vi "Get Tree Items.vi"(8 "Control.Label":string, 9 "VIs.Ctrls":T4[](array[typedef]), 10 "FP.Tr":map{string, T1}(c390), 11 "Data":T6) -> (0 "Used CTRL":bool, 1 "Caption.Visible":bool, 2 "Selected CTRLs":T4[](array[typedef]), 3 "Use in VIs":string[](array[string]), 4 "Tree Items":T7(array[cluster]), 5 "Class Name":T5, 7 "Comment":string)   [LabVIEW 2019, in "Language Editor.lvlib"]
doc: "- - -\nCopyright (c) 2026, Merecs Engineering GmbH"
uses:
  Language Editor.lvlib
  Language Selection/community/Cluster Settings Data.ctl
  type defs/Cluster VI controls.ctl
  type defs/Enum Class Name.ctl
  type defs/Cluster Translations.ctl
  Language Selection/TypeDefs/Cluster PropertyTranslation.ctl
  Language Selection/TypeDefs/Enum Property Type.ctl
  Language Selection/Language Selection.lvlib
panel:
  # "Connector Pane"
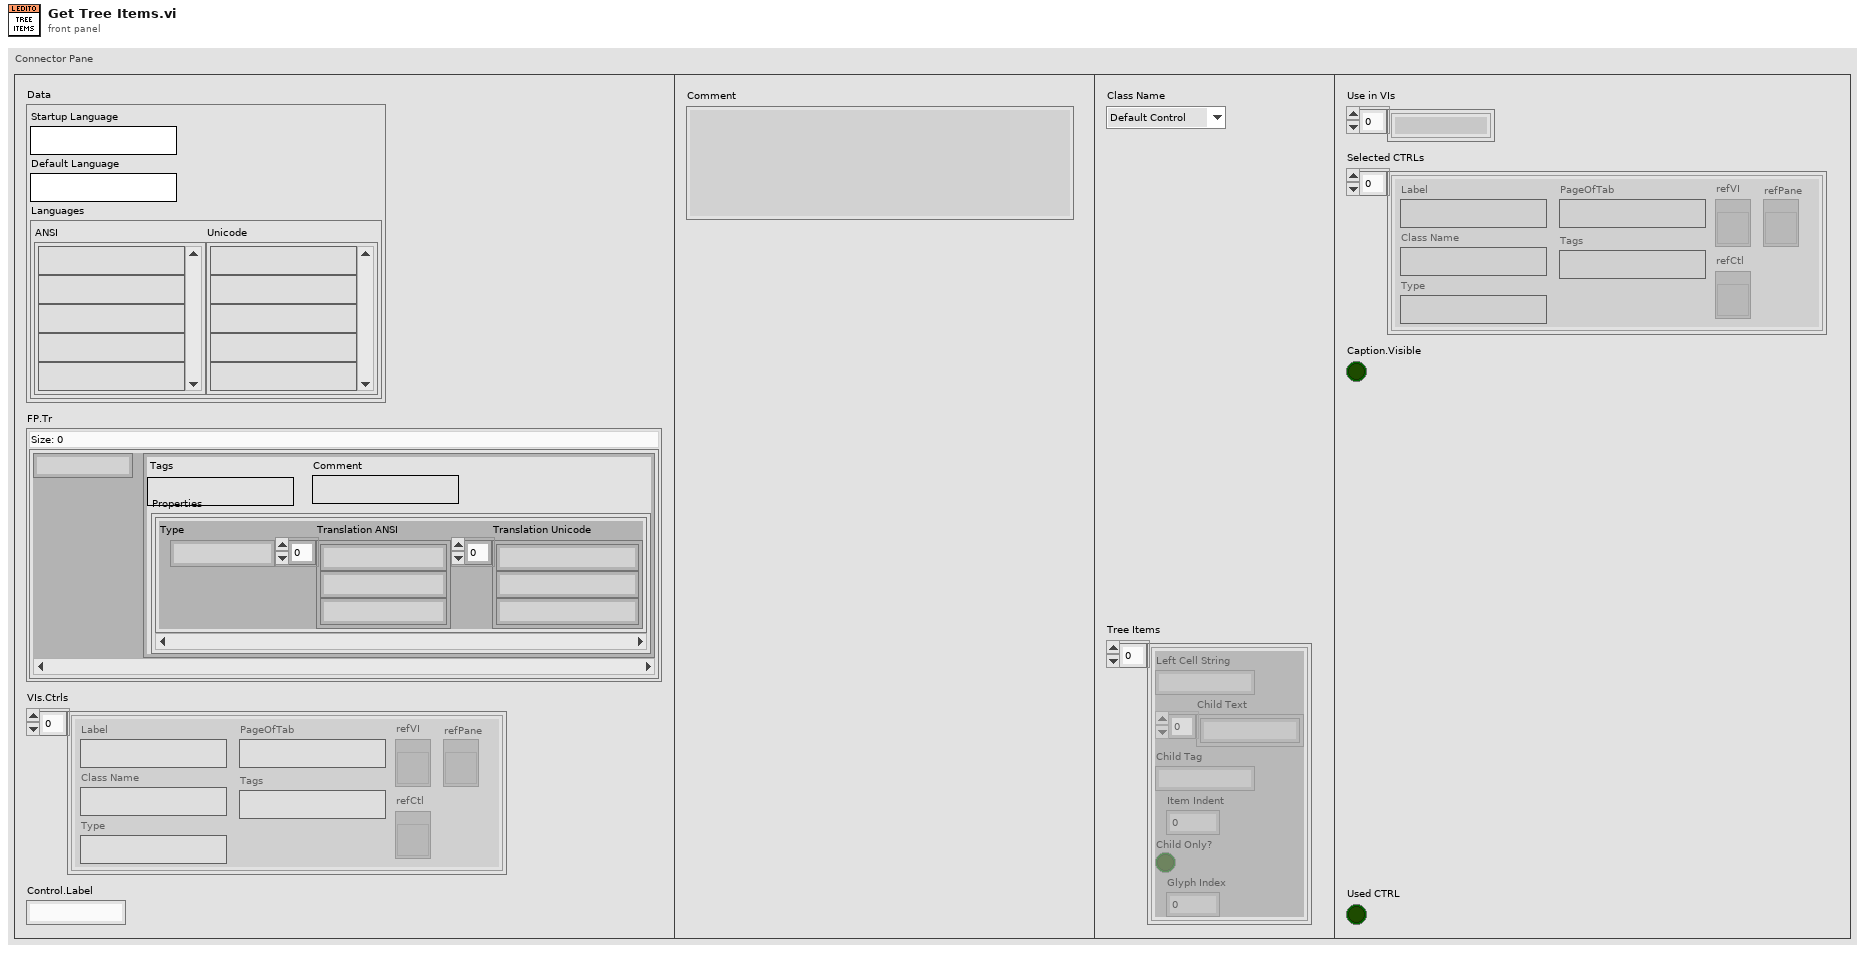
[diagram p1: front panel]
types:
  T1 = typedef "Language Editor.lvlib/Cluster Translations.ctl" = cluster{"Tags":string, "Comment":string, "Properties":T2[]}
  T2 = typedef "Language Selection.lvlib/Cluster PropertyTranslation.ctl" = cluster{"Type":T3, "Translation ANSI":string[], "Translation Unicode":string[]}
  T3 = typedef "Language Selection.lvlib/Enum Property Type.ctl" = enum16{"NA", "Caption", "String Value", "Boolean Text", "Ring Strings", "1D Array Elements", "2D Array Elements", "(MC)Listbox Header", "(MC)Listbox Items", "Tab Pages Names", "X & Y GraphChart", "Plot Names", "Table Headers", "Table Items", "TipStrip", "Combobox Strings", "Cursor Name", "Tree Col Headers"}
  T4 = typedef "Language Editor.lvlib/Cluster VI controls.ctl" = cluster{"Label":string, "Class Name":string, "Type":string, "Tags":string, "refVI":refnum<vi>, "refCtl":refnum<vi>, "PageOfTab":string, "refPane":refnum<vi>}
  T5 = typedef "Language Editor.lvlib/Enum Class Name.ctl" = enum16{"Default Control", "Boolean", "ListBox", "Table", "Graph", "Array", "Ring", "String", "TabControl", "ComboBox", "TreeControl"}
  T6 = typedef "Language Selection.lvlib/Cluster Settings Data.ctl" = cluster{"Startup Language":string, "Default Language":string, "Languages":cluster{"ANSI":string[], "Unicode":string[]}}
  T7 = cluster{"Left Cell String":string, "Child Text":string[], "Child Tag":string, "Item Indent":i32, "Child Only?":bool, "Glyph Index":i32}[]
  T8 = cluster{"Left Cell String":string, "Child Text":string[], "Child Tag":string, "Item Indent":i32, "Child Only?":bool, "Glyph Index":i32}
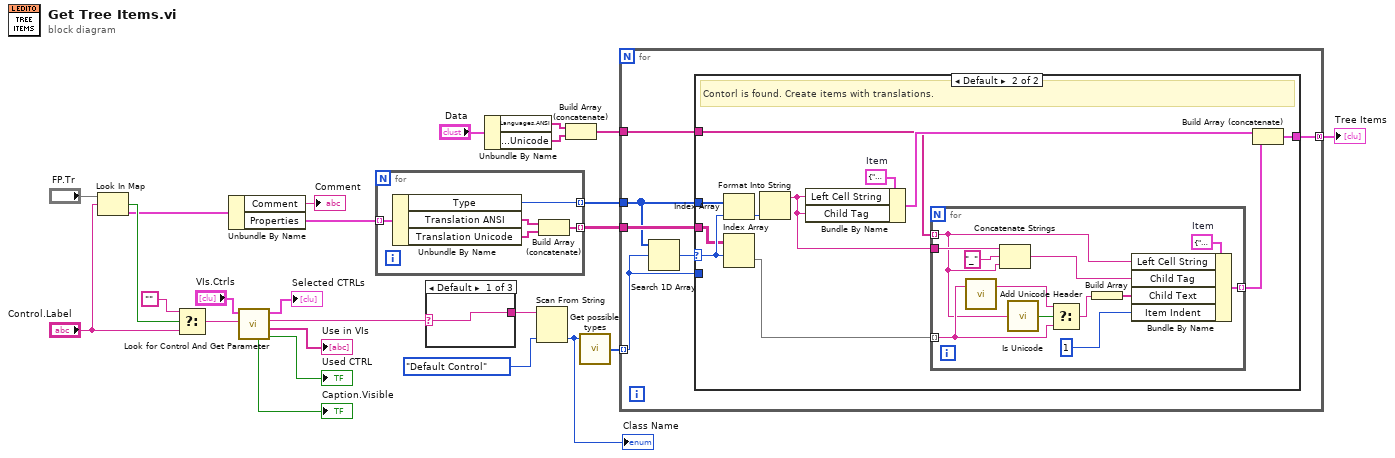
[diagram p0: block diagram]
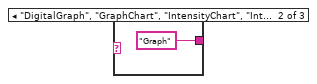
[diagram p2: hidden frame]
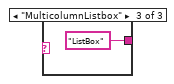
[diagram p3: hidden frame]
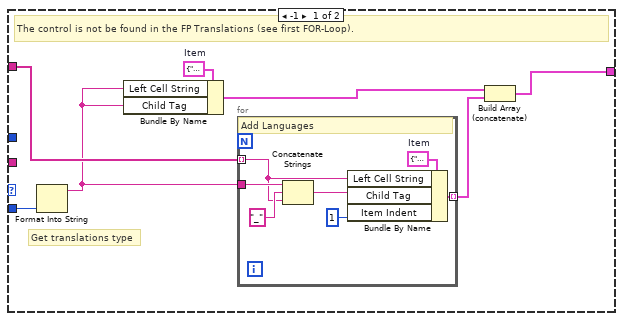
[diagram p4: hidden frame]
diagram:
  n1 = Look In Map(map="FP.Tr", key="Control.Label") -> (key not found?=w5:bool, value=w1:T1)  [unwired: 1 in]
  n2 = Select(t="", s=w5, f="Control.Label") -> (s? t:f=w3:string)
  n3 = Unbundle By Name(w1) -> ("Comment"=→"Comment":string, "Properties"=w15:T2[])
  n4 = call "Look for Control And Get Parameter.vi"("Label"=w3, "VIs.Ctrls"="VIs.Ctrls") -> ("Used CTRL"=→"Used CTRL":bool, "Use in VIs"=→"Use in VIs":string[], "Class Name"=w12:string, "Selected CTRLs"=→"Selected CTRLs":T4[], "Caption Is Vissible"=→"Caption.Visible":bool)  [unwired: 5 in]
  n5 = for {
    tunnel: w15 -> [w30] mode=indexing
    tunnel: [w29] -> w20 mode=indexing
    tunnel: [w26] -> w19 mode=indexing
    n6 = Unbundle By Name(w30) -> ("Type"=w29:T3, "Translation ANSI"=w28:string[], "Translation Unicode"=w27:string[])
    n7 = Build Array (concatenate)(w28, w27) -> (w26:string[])
  }
  n8 = case shown="Default" w12 {
    selector: w12 -> [w31 _ _]
    tunnel: [w31 "Graph" "ListBox"] -> w14
    frame Default {
    }
    frame "DigitalGraph", "GraphChart", "IntensityChart", "IntensityGraph", "MixedSignalGraph", "WaveformChart", "WaveformGraph", "XYGraph" {
    }
    frame "MulticolumnListbox" {
    }
  }
  n9 = Unbundle By Name("Data") -> ("Languages.ANSI"=w23:string[], "Languages.Unicode"=w24:string[])
  n10 = Scan From String(input string=w14, default 1=Enum_Class_Name."Default Control" ("Class Name")) -> (output 1=w25:T5)  [unwired: 3 in, 3 out]
  "Class Name" <- w25
  n11 = Build Array (concatenate)(w23, w24) -> (w18:string[])
  n12 = call "Get possible types.vi"("Class Name"=w25) -> ("Types"=w21:T3[])  [unwired: 4 in]
  n13 = for {
    tunnel: w20 -> [w36]
    tunnel: w19 -> [w38]
    tunnel: w18 -> [w39]
    tunnel: [w37] -> w17 mode=concatenating
    tunnel: w21 -> [w34] mode=indexing
    n14 = Search 1D Array(1D array=w36, element=w34) -> (index of element=w35:i32)  [unwired: 1 in]
    n15 = case shown="Default" w35 {
      selector: w35 -> [_ w64]
      tunnel: w39 -> [w45 w54]
      tunnel: w38 -> [_ w61]
      tunnel: [w42 w58] -> w37
      tunnel: w36 -> [_ w57]
      tunnel: w34 -> [w41 _]
      frame -1 {
        w46 = T8 {"Left Cell String"="", "Child Text"=[], "Child Tag"="", "Item Indent"=0, "Child Only?"=FALSE, "Glyph Index"=0}  # Item
        # "Get translations type"
        # "The control is not be found in the FP Translations (see first FOR-Loop)."
        n16 = Format Into String(w41) -> (resulting string=w40:string)  [unwired: 3 in, 1 out]
        n17 = Bundle By Name(cluster=w46, "Left Cell String"=w40, "Child Tag"=w40) -> (w44:T8)
        n18 = for {
          tunnel: w45 -> [w48] mode=indexing
          tunnel: [w51] -> w43 mode=indexing
          tunnel: w40 -> [w49]
          w53 = T8 {"Left Cell String"="", "Child Text"=[], "Child Tag"="", "Item Indent"=0, "Child Only?"=FALSE, "Glyph Index"=0}  # Item
          # "Add Languages"
          n19 = Concatenate Strings(w49, "_" ("string"), w48) -> (w47:string)
          n20 = Bundle By Name(cluster=w53, "Left Cell String"=w48, "Child Tag"=w47, "Item Indent"=1) -> (w51:T8)
        }
        n21 = Build Array (concatenate)(w44, w43) -> (w42:T7)
      }
      frame Default {
        w62 = T8 {"Left Cell String"="", "Child Text"=[], "Child Tag"="", "Item Indent"=0, "Child Only?"=FALSE, "Glyph Index"=0}  # Item
        # "Contorl is found. Create items with translations."
        n22 = Index Array(array=w57, index=w64) -> (element=w63:T3)
        n23 = Index Array(array=w61, index (row)=w64) -> (element=w56:string[])  [unwired: 1 in]
        n24 = Format Into String(w63) -> (resulting string=w55:string)  [unwired: 3 in, 1 out]
        n25 = Bundle By Name(cluster=w62, "Left Cell String"=w55, "Child Tag"=w55) -> (w60:T8)
        n26 = for {
          tunnel: w54 -> [w65] mode=indexing
          tunnel: w56 -> [w72] mode=indexing
          tunnel: [w69] -> w59 mode=indexing
          tunnel: w55 -> [w68]
          w76 = T8 {"Left Cell String"="", "Child Text"=[], "Child Tag"="", "Item Indent"=0, "Child Only?"=FALSE, "Glyph Index"=0}  # Item
          n27 = call "Add Unicode Header.vi"("Text"=w72) -> ("Text with header"=w74:string)  [unwired: 1 in, 1 out]
          n28 = Concatenate Strings(w68, "_" ("string"), w65) -> (w66:string)
          n29 = call "Is Unicode.vi"("Language"=w65) -> ("Is Unicode"=w73:bool)
          n30 = Select(t=w74, s=w73, f=w72) -> (s? t:f=w71:string)
          n31 = Build Array(w71) -> (w70:string[])
          n32 = Bundle By Name(cluster=w76, "Left Cell String"=w65, "Child Tag"=w66, "Child Text"=w70, "Item Indent"=1) -> (w69:T8)
        }
        n33 = Build Array (concatenate)(w60, w59) -> (w58:T7)
      }
    }
  }
  "Tree Items" <- w17
